vi "RDC-compare_deembed.vi"() -> ()   [LabVIEW 2020]
doc: "Compares de-embedding results, run by hand. It reads common-format files, applies the propagation-constant and reflection corrections, computes impedance and coax length, and shows the results on Smith plots."
uses:
  RDC-dielectric_types.ctl
  Reflector/RFH-Reflection_File_Handler.lvlib
  RDC-Reflection_Data_Computation.lvlib
panel:
  out "lenght array":dbl[][](graph)
  in  "Autoscale 2":bool=TRUE
  out "Smith Plot 9":picture
  out "Smith Plot 8":picture
  out "Smith Plot 7":picture
  out "Smith Plot 6":picture
  out "Smith Plot 5":picture
  out "Smith Plot 4":picture
  in  "Autoscale":bool=TRUE
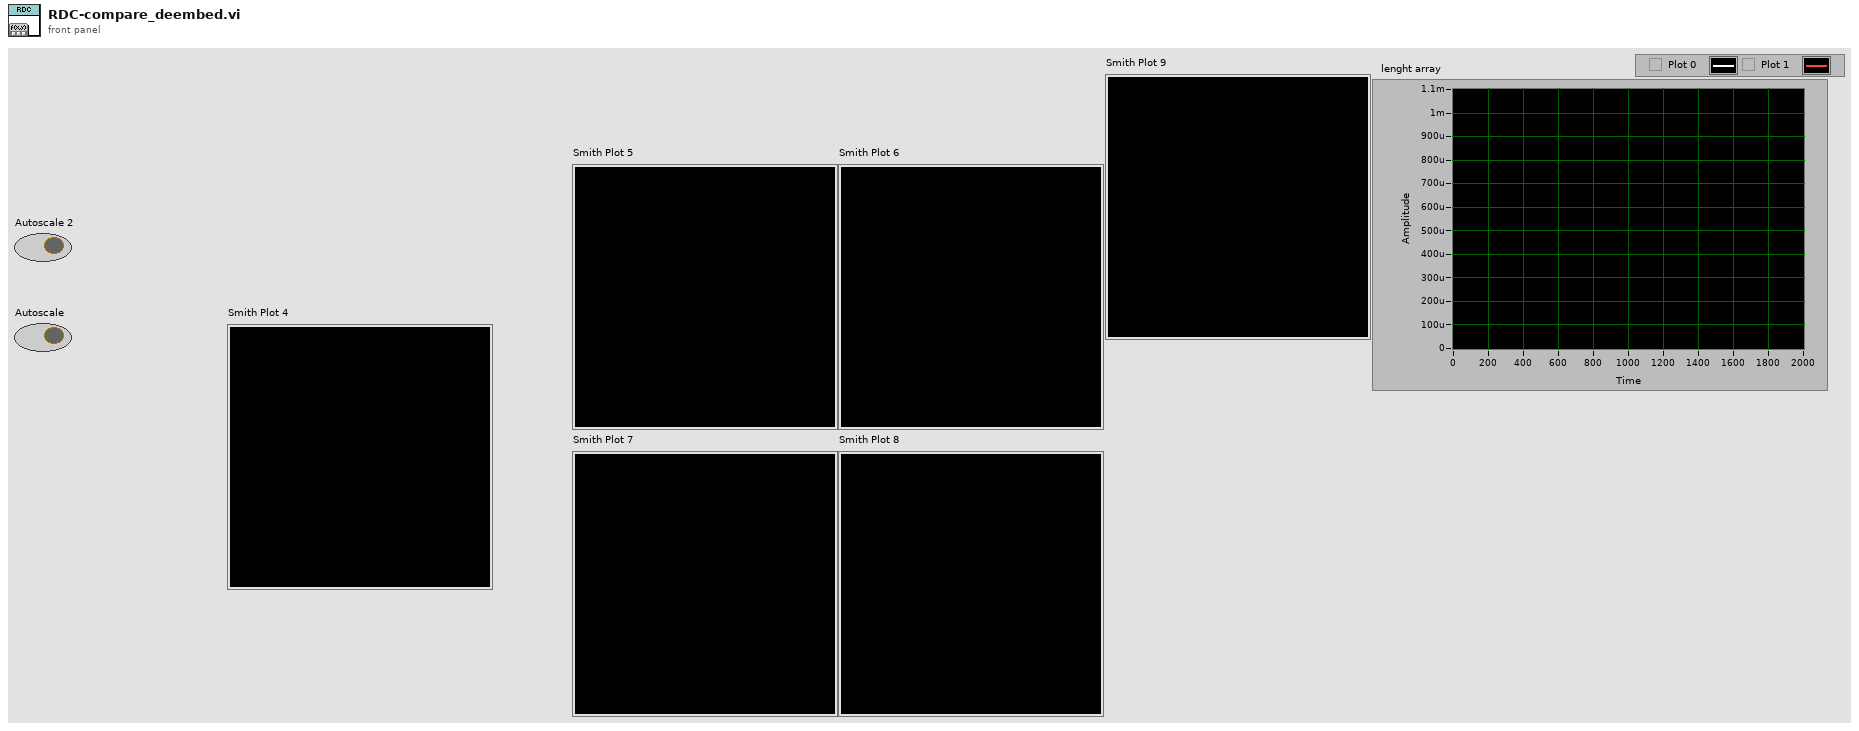
[diagram p1: front panel]
types:
  T1 = typedef "RDC-Reflection_Data_Computation.lvlib/RDC-dielectric_types.ctl" = enum16{"Teflon", "Eccostock 0005"}
  T2 = cluster{"x minimum":dbl, "x maximum":dbl, "y minimum":dbl, "y maximum":dbl}
  T3 = typedef "RFH-Reflection_File_Handler.lvlib/RFH-common_data_format.ctl" = cluster{"Frequency":dbl[], "Reflection'":dbl[], "Reflection''":dbl[], "Permativity'":dbl[], "Permativity''":dbl[], "Conductivity":dbl[], "Loss Tangent":dbl[], "Resistance":dbl[], "Reactance":dbl[]}
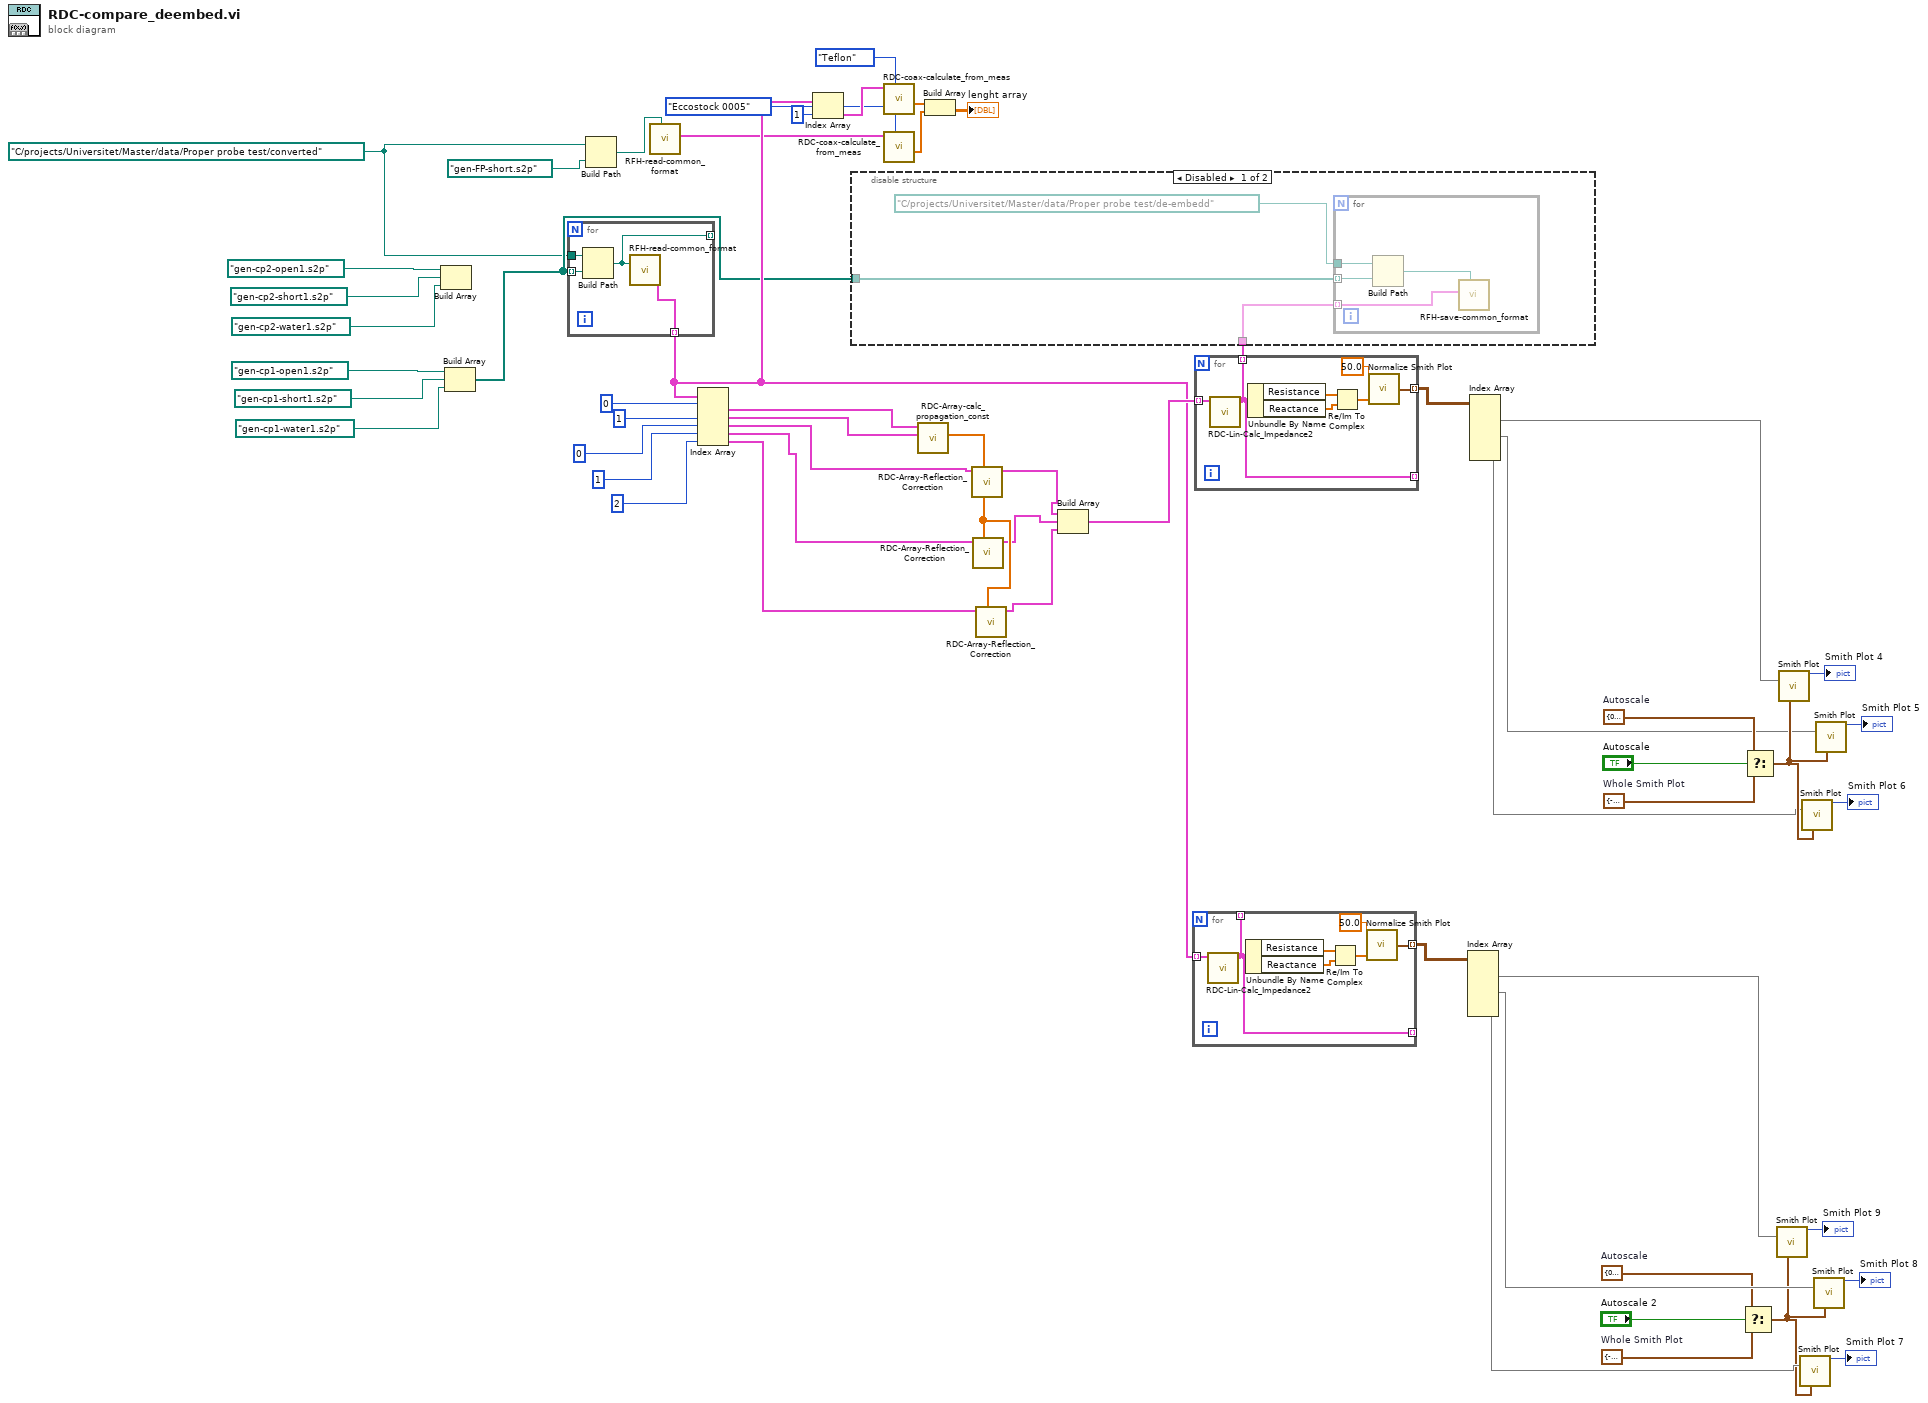
[diagram p0: block diagram]
diagram:
  w20 = T2 {"x minimum"=0.0, "x maximum"=0.0, "y minimum"=0.0, "y maximum"=0.0}  # Autoscale
  w18 = T2 {"x minimum"=-1.0, "x maximum"=1.0, "y minimum"=-1.0, "y maximum"=1.0}  # Whole Smith Plot
  w37 = T2 {"x minimum"=0.0, "x maximum"=0.0, "y minimum"=0.0, "y maximum"=0.0}  # Autoscale
  w39 = T2 {"x minimum"=-1.0, "x maximum"=1.0, "y minimum"=-1.0, "y maximum"=1.0}  # Whole Smith Plot
  w8 = path "C:/projects/Universitet/Master/data/Proper probe test/converted" ("base path")
  n1 = Build Array(path "gen-cp2-open1.s2p" ("file path (dialog if empty)"), path "gen-cp2-short1.s2p" ("file path (dialog if empty)"), path "gen-cp2-water1.s2p" ("file path (dialog if empty)")) -> ()  [unwired: 1 out]
  n2 = Build Array(path "gen-cp1-open1.s2p" ("file path (dialog if empty)"), path "gen-cp1-short1.s2p" ("file path (dialog if empty)"), path "gen-cp1-water1.s2p" ("file path (dialog if empty)")) -> (w10:path[])
  n3 = for {
    tunnel: w8 -> [w61]
    tunnel: [w60] -> w16 mode=indexing
    tunnel: [w59] -> _ mode=indexing
    tunnel: w10 -> [w58] mode=indexing
    n4 = Build Path(base path=w61, name or relative path=w58) -> (appended path=w59:path)
    n5 = call "RFH-read-common_format.vi"("file path (dialog if empty)"=w59) -> ("Common Format"=w60:T3)  [unwired: 9 in, 1 out]
  }
  n6 = Build Path(base path=w8, name or relative path=path "gen-FP-short.s2p" ("file path (dialog if empty)")) -> (appended path=w7:path)
  n7 = call "RFH-read-common_format.vi"("file path (dialog if empty)"=w7) -> ("Common Format"=w6:T3)  [unwired: 9 in, 1 out]
  n8 = Index Array(array=w16, index #1=0 ("index"), index #2=1 ("index"), index #3=0 ("index"), index #4=1 ("index"), index #5=2 ("index")) -> (element #1=w50:T3, element #2=w49:T3, element #3=w48:T3, element #4=w47:T3, element #5=w46:T3)
  n9 = Index Array(array=w16, index=1) -> (element=w15:T3)
  n10 = call "RDC-coax-calculate_from_meas.vi"("dielectric"=RDC-dielectric_types."Teflon", "measurement"=w15) -> ("lenght array"=w3:dbl[])  [unwired: 7 in, 2 out]
  n11 = call "RDC-coax-calculate_from_meas.vi"("dielectric"=RDC-dielectric_types."Eccostock 0005", "measurement"=w6) -> ("lenght array"=w1:dbl[])  [unwired: 7 in, 2 out]
  n12 = call "RDC-Array-calc_propagation_const.vi"("Measured open"=w49, "Measured Short"=w50) -> ("e gamma mix"=w54:cdb[])  [unwired: 8 in, 1 out]
  n13 = Build Array(w3, w1) -> (→"lenght array":dbl[][])
  n14 = call "RDC-Array-Reflection_Correction.vi"("e gamma mix"=w54, "Measured"=w48) -> ("Tip"=w41:T3)  [unwired: 8 in, 1 out]
  n15 = call "RDC-Array-Reflection_Correction.vi"("e gamma mix"=w54, "Measured"=w47) -> ("Tip"=w42:T3)  [unwired: 8 in, 1 out]
  n16 = call "RDC-Array-Reflection_Correction.vi"("e gamma mix"=w54, "Measured"=w46) -> ("Tip"=w40:T3)  [unwired: 8 in, 1 out]
  n17 = Build Array(w41, w42, w40) -> (w29:T3[])
  n18 = for {
    tunnel: [w64] -> w17 mode=indexing
    tunnel: [w62] -> _ mode=indexing
    tunnel: w16 -> [w63] mode=indexing
    tunnel: [w62] -> _ mode=indexing
    n19 = call "RDC-Lin-Calc_Impedance2.vi"("input cluster"=w63) -> ("Output cluster"=w62:T3)  [unwired: 9 in, 1 out]
    n20 = Unbundle By Name(w62) -> ("Resistance"=w67:dbl[], "Reactance"=w66:dbl[])
    n21 = Re/Im To Complex(1:w66, 2:w67) -> (0:w65:cdb[])
    n22 = call <vilib>:"Normalize Smith Plot.vi"("points complex"=w65, "Zo (50.0)"=50.0) -> ("normalized smith points {r,x}"=w64:cluster{"r":dbl, "x":dbl}[])  [unwired: 1 in]
  }
  n23 = for {
    tunnel: [w71] -> w53 mode=indexing
    tunnel: [w69] -> _ mode=indexing
    tunnel: w29 -> [w70] mode=indexing
    tunnel: [w69] -> w28 mode=indexing
    n24 = call "RDC-Lin-Calc_Impedance2.vi"("input cluster"=w70) -> ("Output cluster"=w69:T3)  [unwired: 9 in, 1 out]
    n25 = Unbundle By Name(w69) -> ("Resistance"=w74:dbl[], "Reactance"=w73:dbl[])
    n26 = Re/Im To Complex(1:w73, 2:w74) -> (0:w72:cdb[])
    n27 = call <vilib>:"Normalize Smith Plot.vi"("points complex"=w72, "Zo (50.0)"=50.0) -> ("normalized smith points {r,x}"=w71:cluster{"r":dbl, "x":dbl}[])  [unwired: 1 in]
  }
  n28 = disable-structure shown="Disabled" {
    disable-tunnel: w28 -> [w78 _]
    disable-tunnel: w10 -> [w76 _]
    frame Disabled {
      n29 = for {
        tunnel: w78 -> [w79] mode=indexing
        tunnel: path "C:/projects/Universitet/Master/data/Proper probe test/de-embedd" ("base path") -> [w82]
        tunnel: w76 -> [w81] mode=indexing
        n30 = Build Path(base path=w82, name or relative path=w81) -> (appended path=w80:path)
        n31 = call "RFH-save-common_format.vi"("file path (use dialog)"=w80, "Common Format"=w79) -> ()  [unwired: 9 in, 1 out]
      }
    }
    frame Enabled {
    }
  }
  n32 = Index Array(array=w17) -> (element #1=w22:cluster{"r":dbl, "x":dbl}[], element #2=w26:cluster{"r":dbl, "x":dbl}[], element #3=w27:cluster{"r":dbl, "x":dbl}[])  [unwired: 6 in]
  n33 = Index Array(array=w53) -> (element #1=w35:cluster{"r":dbl, "x":dbl}[], element #2=w31:cluster{"r":dbl, "x":dbl}[], element #3=w30:cluster{"r":dbl, "x":dbl}[])  [unwired: 6 in]
  n34 = Select(t=w20, s="Autoscale 2", f=w18) -> (s? t:f=w25:T2)
  n35 = Select(t=w37, s="Autoscale", f=w39) -> (s? t:f=w32:T2)
  n36 = call <vilib>:"Smith Plot.vi"("smith plot"=w22, "smith plot section"=w25) -> ("new picture"=→"Smith Plot 9":picture)  [unwired: 13 in]
  n37 = call <vilib>:"Smith Plot.vi"("smith plot"=w35, "smith plot section"=w32) -> ("new picture"=→"Smith Plot 4":picture)  [unwired: 13 in]
  n38 = call <vilib>:"Smith Plot.vi"("smith plot"=w27, "smith plot section"=w25) -> ("new picture"=→"Smith Plot 7":picture)  [unwired: 13 in]
  n39 = call <vilib>:"Smith Plot.vi"("smith plot"=w30, "smith plot section"=w32) -> ("new picture"=→"Smith Plot 6":picture)  [unwired: 13 in]
  n40 = call <vilib>:"Smith Plot.vi"("smith plot"=w26, "smith plot section"=w25) -> ("new picture"=→"Smith Plot 8":picture)  [unwired: 13 in]
  n41 = call <vilib>:"Smith Plot.vi"("smith plot"=w31, "smith plot section"=w32) -> ("new picture"=→"Smith Plot 5":picture)  [unwired: 13 in]
